vi "Ask User.vi"(8 "error in":errorcluster, 9 "requestedSchema":string, 10 "message":string, 11 "key":string) -> (0 "error out":errorcluster, 2 "content":string, 3 "action":T1(ring))   [LabVIEW 2020, in "MCP Server.lvlib"]
doc: "Asks the user of the MCP client a question while a tool runs (MCP elicitation, form mode), using the multi round-trip pattern of MCP 2026-07-28: the tool VI runs twice. On the first run the question is only registered and action is \"pending\"; tools/call then answers the client with resultType \"input_required\". The client shows the question and calls the tool again with the user's answer, and on that second run action is accept, decline or cancel and content holds the answer.\n\nHOW TO USE IT IN A TOOL VI: call Ask User.vi before doing anything that has side effects. When action is \"pending\", return at once and do NOTHING else (no hardware access, no file writes): the run is thrown away and the tool runs again with the answer. Do the real work only on the run that has the answer (accept), and handle decline and cancel. When action is \"not supported\", the client cannot be asked (a legacy client, or a client without the elicitation capability): fall back to a safe default or refuse, and say so in the tool's outputs.\n\nkey identifies the question and must be unique within the tool (use a fixed text such as \"confirm_delete\"); several questions need several keys.\n\nrequestedSchema is passed to the client as given. MCP restricts it to a flat object whose properties are primitives only: string (minLength, maxLength, format email/uri/date/date-time, default), number or integer (minimum, maximum, default), boolean (default) and enums of strings, each with optional title and description. Empty means a plain confirmation, {\"type\":\"object\",\"properties\":{}}; anything that is not a JSON object is replaced by that too. Form mode MUST NOT be used to ask for passwords, API keys, tokens or other secrets.\n\nOnly works inside tools/call of a modern request (params._meta with io.modelcontextprotocol/protocolVersion) whose client declared the elicitation capability ({} counts as form mode). The request context comes from Handle MCP Request.vi through the named queues \"MCP Request Context\" and \"MCP Input Requests\". Legacy requests always get \"not supported\": legacy elicitation needs a server-to-client stream, which this server does not have."
uses:
  MCP Server.lvlib
  <vilib>/JDP Science/JSONtext/LVClass Serializer/JSONtext LVClass Serializer.lvclass
  <vilib>/JDP Science/JSONtext/JSONtext.lvlib
  124ded27-594c-4037-bf2e-379795ac4b2e.vi
  62da56eb-f0a6-4b80-a83c-1ca9a1e03e4a.vi
  2fef378c-373f-410f-8824-e3c99f95a5c8.vi
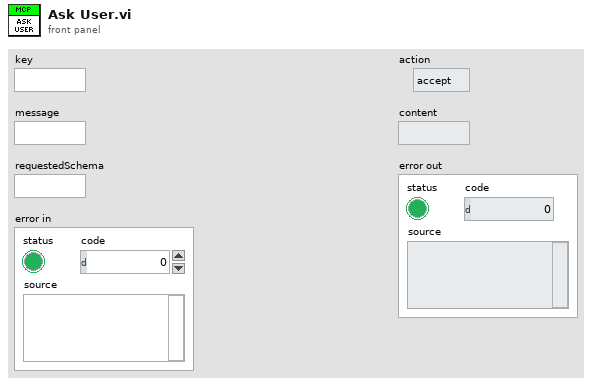
[diagram p1: front panel]
types:
  T1 = enum16{"accept", "decline", "cancel", "pending", "not supported"}
  T2 = enum16{"accept", "decline", "cancel", "pending", "not supported"}[]
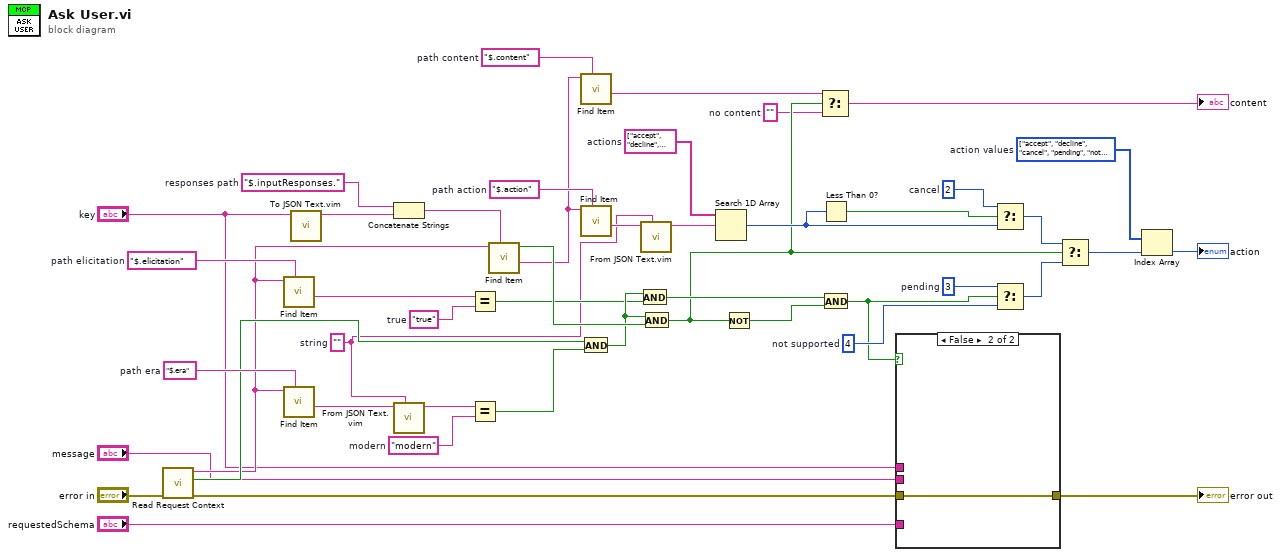
[diagram p0: block diagram]
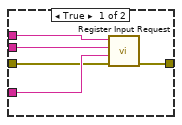
[diagram p2: hidden frame]
diagram:
  w9 = ""  # no content
  w15 = T2 [enum."accept", enum."decline", enum."cancel", enum."pending", enum."not supported"] items=["accept", "decline", "cancel", "pending", "not supported"]  # action values
  w18 = 4  # not supported
  w19 = 3  # pending
  w22 = 2  # cancel
  w24 = string[] ["accept", "decline", "cancel"]  # actions
  w12 = "$.content"  # path content
  w27 = "$.action"  # path action
  w36 = "$.inputResponses."  # responses path
  w37 = "true"  # true
  w39 = "$.elicitation"  # path elicitation
  w42 = "modern"  # modern
  w25 = ""  # string
  w45 = "$.era"  # path era
  n1 = call "Read Request Context.vi"("error in"="error in") -> ("error out"=w5:errorcluster, "found?"=w41:bool, "context"=w34:string)  [unwired: 8 in]
  n2 = call <vilib>:"Find Item.vi"("$Path or Item Name"=w39, "JSON"=w34) -> ("<JSON>"=w38:string)  [unwired: 6 in, 3 out]
  n3 = call <vilib>:"Find Item.vi"("$Path or Item Name"=w45, "JSON"=w34) -> ("<JSON>"=w44:string)  [unwired: 6 in, 3 out]
  n4 = call "To JSON Text.vim"("Anything"="key") -> ("<JSON>"=w35:string)  [unwired: 9 in, 1 out]
  n5 = Concatenate Strings(w36, w35) -> (w33:string)
  n6 = call "From JSON Text.vim"("Data Type and Default Value"=w25, "JSON"=w44) -> ("Data out"=w43:string)  [unwired: 8 in, 1 out]
  n7 = Equal?(x=w38, y=w37) -> (x = y?=w30:bool)
  n8 = Equal?(x=w43, y=w42) -> (x = y?=w40:bool)
  n9 = call <vilib>:"Find Item.vi"("$Path or Item Name"=w33, "JSON"=w34) -> ("<JSON>"=w13:string, "Found"=w32:bool)  [unwired: 6 in, 2 out]
  n10 = call <vilib>:"Find Item.vi"("$Path or Item Name"=w12, "JSON"=w13) -> ("<JSON>"=w11:string)  [unwired: 6 in, 3 out]
  n11 = call <vilib>:"Find Item.vi"("$Path or Item Name"=w27, "JSON"=w13) -> ("<JSON>"=w26:string)  [unwired: 6 in, 3 out]
  n12 = And(x=w41, y=w40) -> (x .and. y?=w31:bool)
  n13 = And(x=w31, y=w30) -> (x .and. y?=w29:bool)
  n14 = call "From JSON Text.vim"("Data Type and Default Value"=w25, "JSON"=w26) -> ("Data out"=w23:string)  [unwired: 8 in, 1 out]
  n15 = And(x=w31, y=w32) -> (x .and. y?=w10:bool)
  n16 = Search 1D Array(1D array=w24, element=w23) -> (index of element=w20:i32)  [unwired: 1 in]
  n17 = Not(x=w10) -> (.not. x?=w28:bool)
  n18 = Select(t=w11, s=w10, f=w9) -> (s? t:f=→"content":string)
  n19 = Less Than 0?(x=w20) -> (x < 0?=w21:bool)
  n20 = And(x=w29, y=w28) -> (x .and. y?=w4:bool)
  n21 = case shown="False" w4 {
    tunnel: "key" -> [w51 _]
    tunnel: "message" -> [w50 _]
    tunnel: "requestedSchema" -> [w49 _]
    tunnel: w5 -> [w48 w52]
    tunnel: [w47 w52] -> w1
    frame True {
      n22 = call "Register Input Request.vi"("error in"=w48, "requestedSchema"=w49, "message"=w50, "key"=w51) -> ("error out"=w47:errorcluster)  [unwired: 7 in]
    }
    frame False {
    }
  }
  "error out" <- w1
  n23 = Select(t=w22, s=w21, f=w20) -> (s? t:f=w17:i32)
  n24 = Select(t=w19, s=w4, f=w18) -> (s? t:f=w16:i32)
  n25 = Select(t=w17, s=w10, f=w16) -> (s? t:f=w14:i32)
  n26 = Index Array(array=w15, index=w14) -> (element=→"action":T1)
